vi "Main (429).vi"() -> ()   [LabVIEW 2023]
doc: "Use this template to build a simple state machine design pattern. Each state executes code and determines which state to transition to."
uses:
  Controls/State.ctl
  Controls/Data.ctl
  Controls/Database_Array.ctl
  Controls/Encoding.ctl
  <vilib>/Utility/error.llb/DialogType.ctl
  <userlib>/_OpenG.lib/array/array.llb/Remove Duplicates from 1D Array (I32)__ogtk.vi
  <userlib>/_OpenG.lib/array/array.llb/Sort 1D Array (I32)__ogtk.vi
  <userlib>/_OpenG.lib/array/array.llb/Search 1D Array (I32)__ogtk.vi
  <userlib>/_OpenG.lib/array/array.llb/Index 1D Array Elements (Variant)__ogtk.vi
  Libraries/Ballard_429_Parameter_ni/Ballard_429_Parameter_ni.lvlib
  Libraries/Aim_429_Parameter_ni/AIM_429_Parameter_ni.lvlib
panel:
  in  "Enable Large Schedules?":bool
  in  "Create Timestamp Channels?":bool
  in  "Use Octal Labels?":bool
  in  "formatting":enum16{"NIVeriStandAdd-Ons", "ni", "ni-AIM"}(ring)
  in  "Configure SelfTestBus?":bool
  out "Progress":string
  in  "Stop Button":bool
  in  "Generate XMLs":bool
  in  "Database Filepath (xlsx)":path
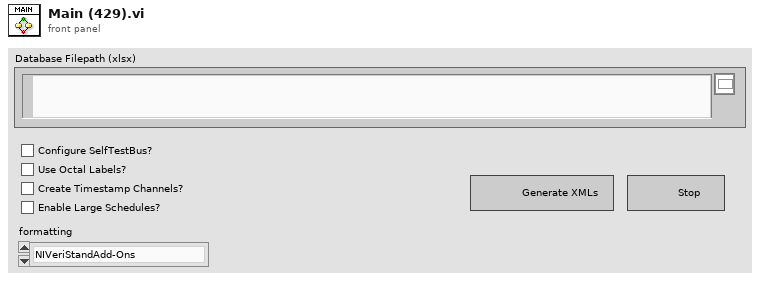
[diagram p1: front panel]
types:
  T1 = typedef "DialogType.ctl" = u16
  T2 = typedef "Data.ctl" = cluster{"Cores to Process Array":i32[], "All Parameters Array":T3[], "Filtered Parameter Array":T3[], "Core Number":i32, "Database Filepath (xlsx)":path, "Selected Self Test Channels":i32[], "formatting":enum16{"NIVeriStandAdd-Ons", "ni", "ni-AIM"}, "Use Octal Labels?":bool, "Create Timestamp Channels?":bool, "Configure SelfTestBus?":bool, "Enable Large Schedules?":bool}
  T3 = typedef "Database_Array.ctl" = cluster{"Core Number":i32, "Channel Number":i32, "Channel Name":string, "Channel Speed":i32, "Label Decimal":u32, "Label Name":string, "Min Rate (mS)":i32, "Max Rate (mS)":i32, "SDI":i32, "SSM":i32, "Create SDI":bool, "Create SSM":bool, "Create Parity":bool, "Parameter Name":string, "Start Bit":i32, "Number of Bits":i32, "Scale":string, "Offset":string, "Signed":bool, "Unit":string, "Encoding":T4, "Default Value":string}
  T4 = typedef "Encoding.ctl" = enum16{"BCD", "BNR", "Discrete"}
  T5 = typedef "State.ctl" = enum16{"Initialize", "Wait for Event", "Read Database File", "Get Core Data", "Write HW XML File", "Write Parameter XML File", "Exit"}
  T6 = enum8{"Enabled", "Disabled", "Disabled and Grayed Out"}
  T7 = enum32{"invalid app kind", "Development System", "Run Time System", "Student Edition", "Embedded LabVIEW", "Evaluation", "Custom"}
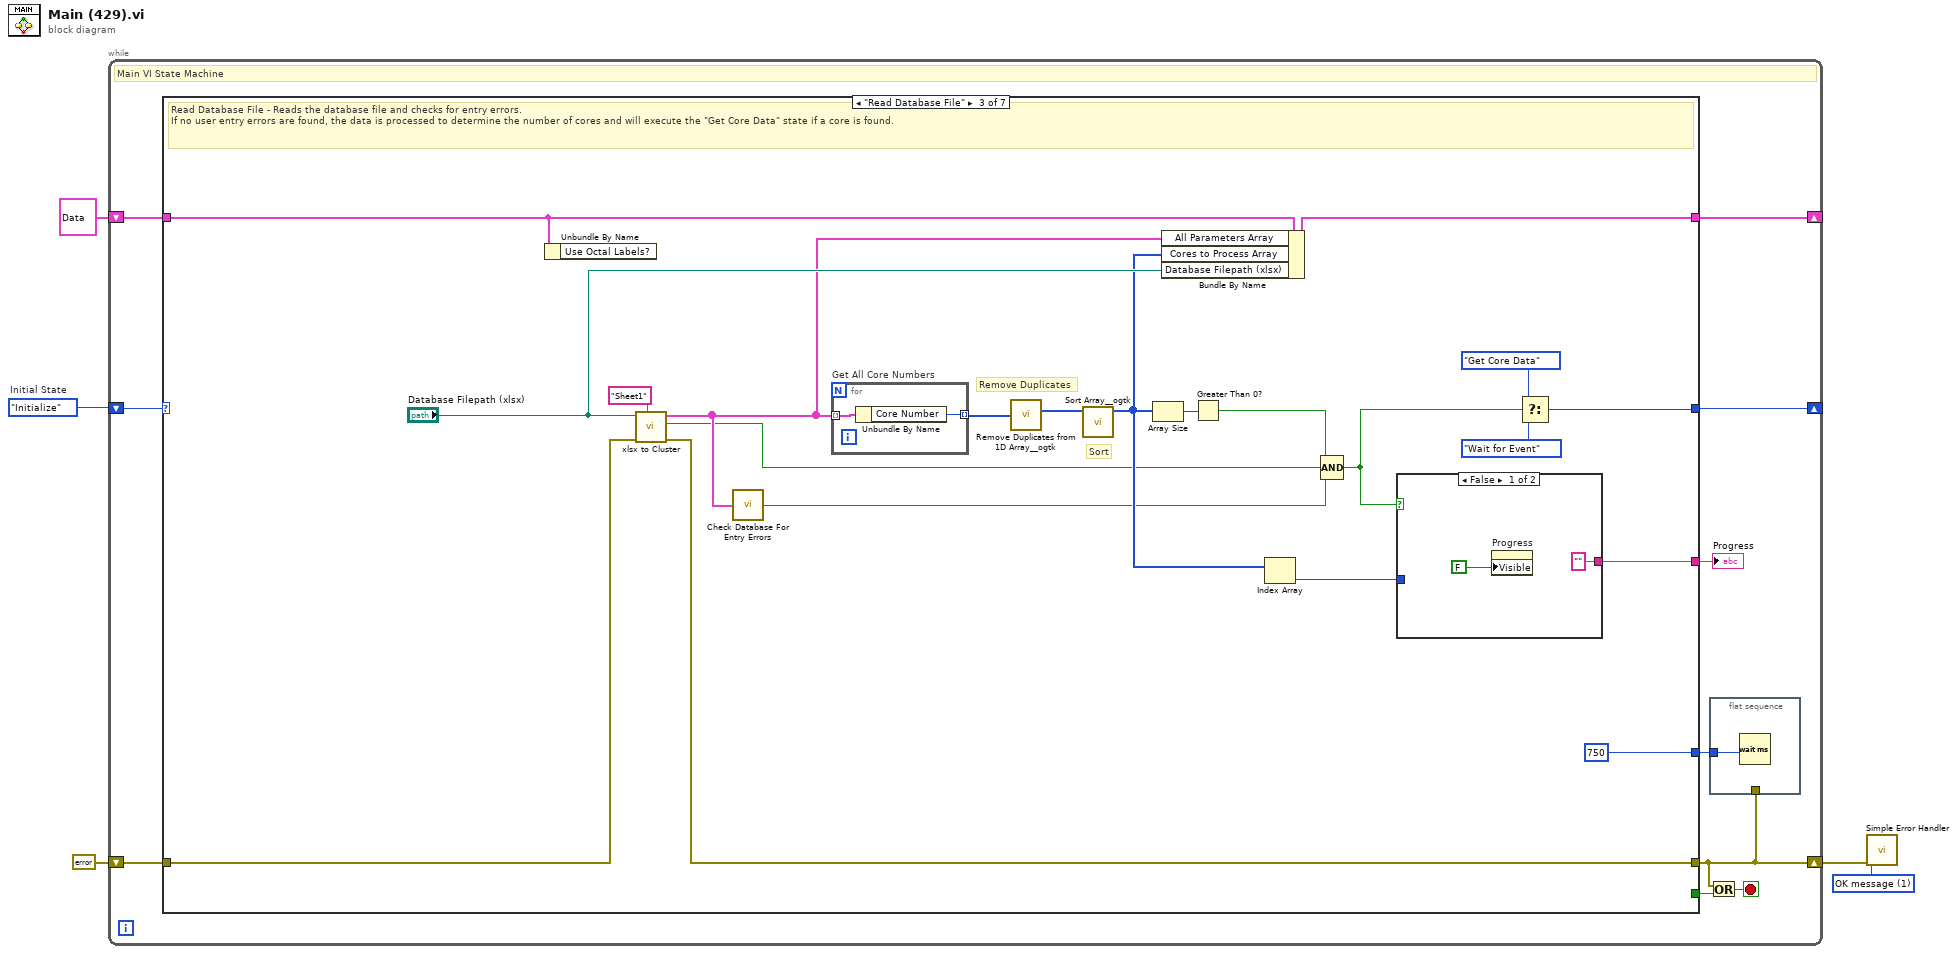
[diagram p0: block diagram]
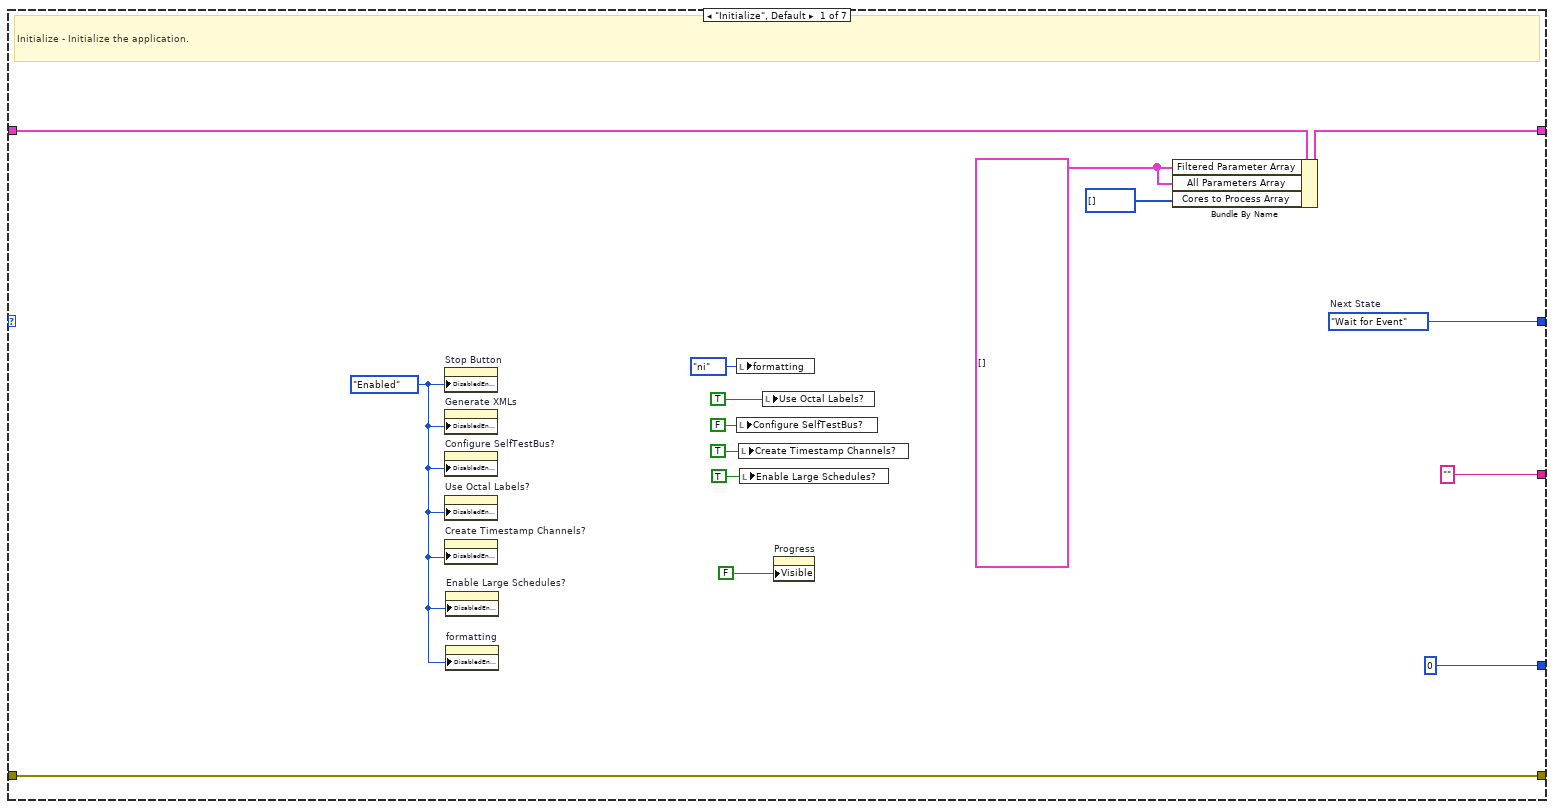
[diagram p2: hidden frame]
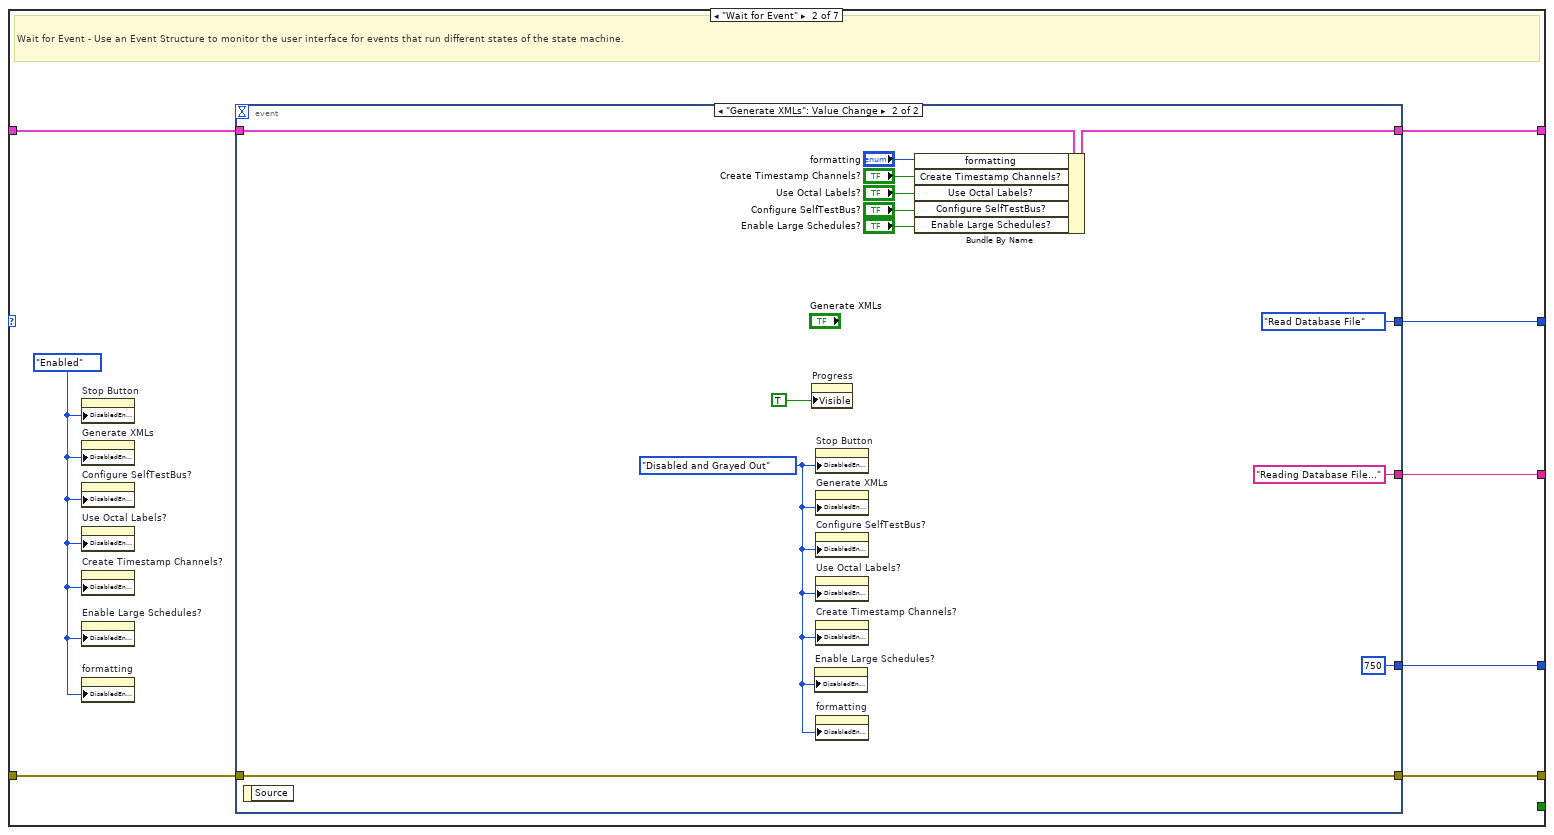
[diagram p3: hidden frame]
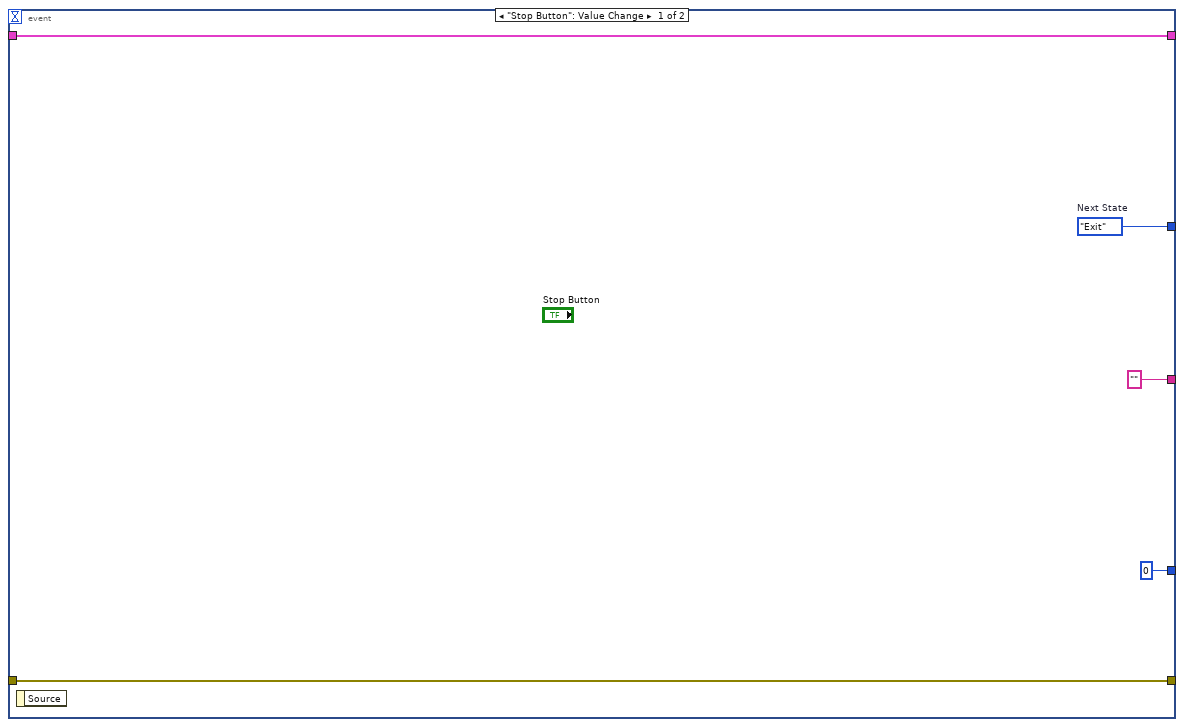
[diagram p4: hidden frame]
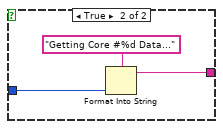
[diagram p5: hidden frame]
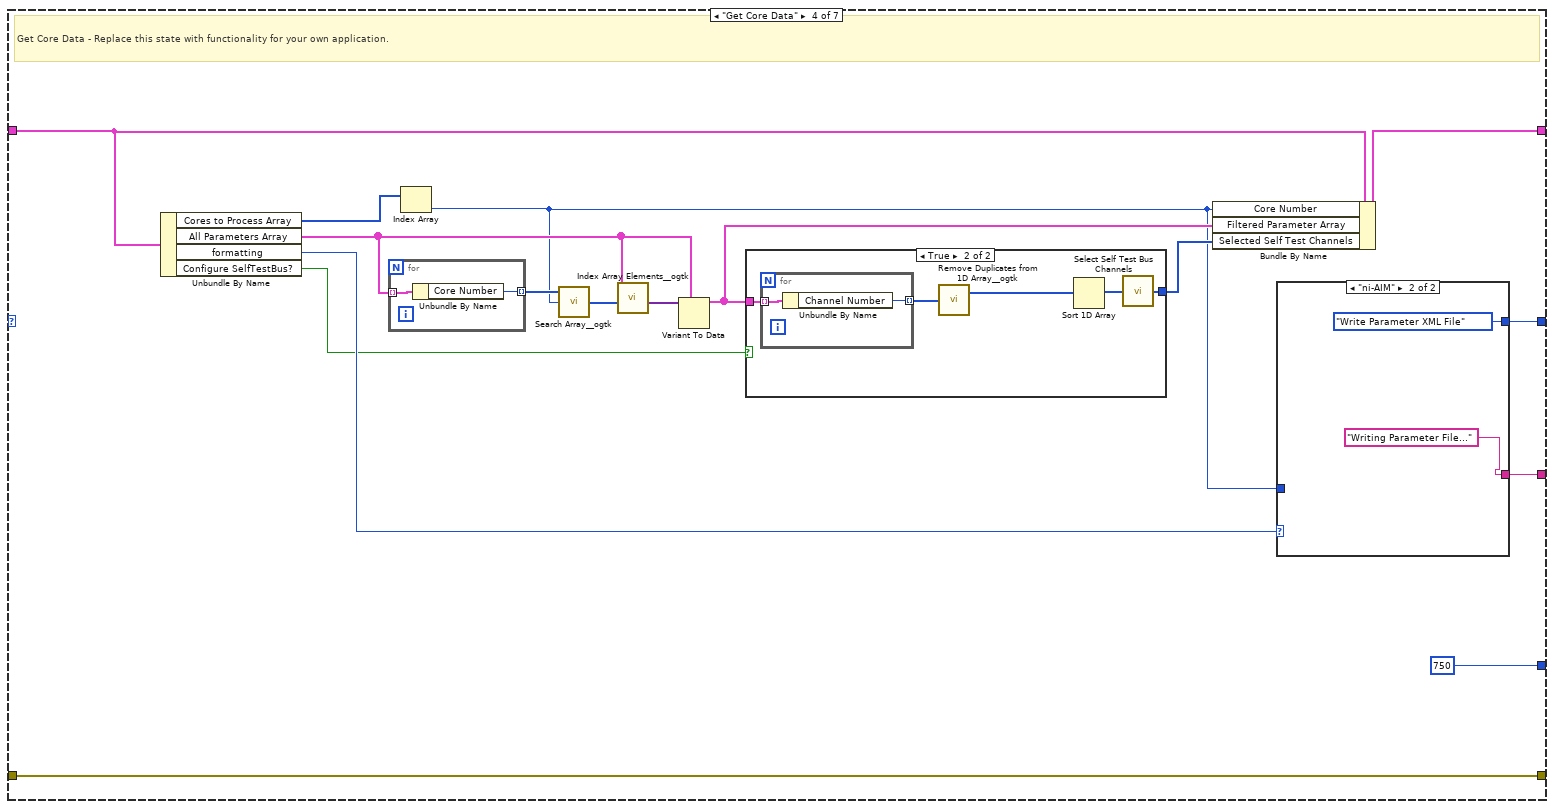
[diagram p6: hidden frame]
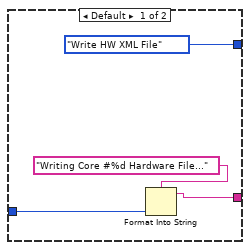
[diagram p7: hidden frame]
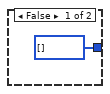
[diagram p8: hidden frame]
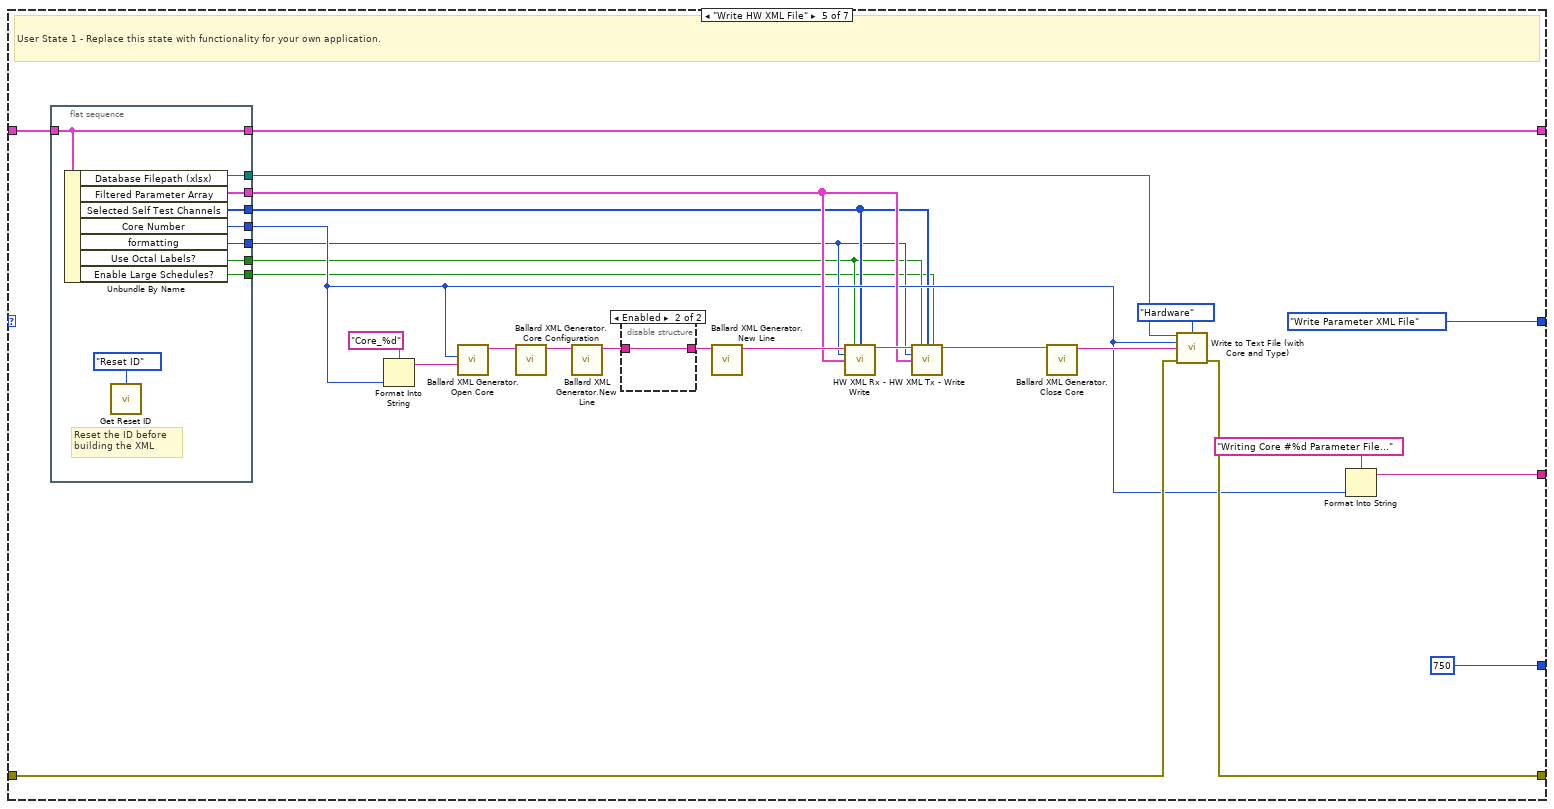
[diagram p9: hidden frame]
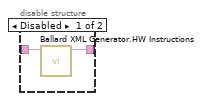
[diagram p10: hidden frame]
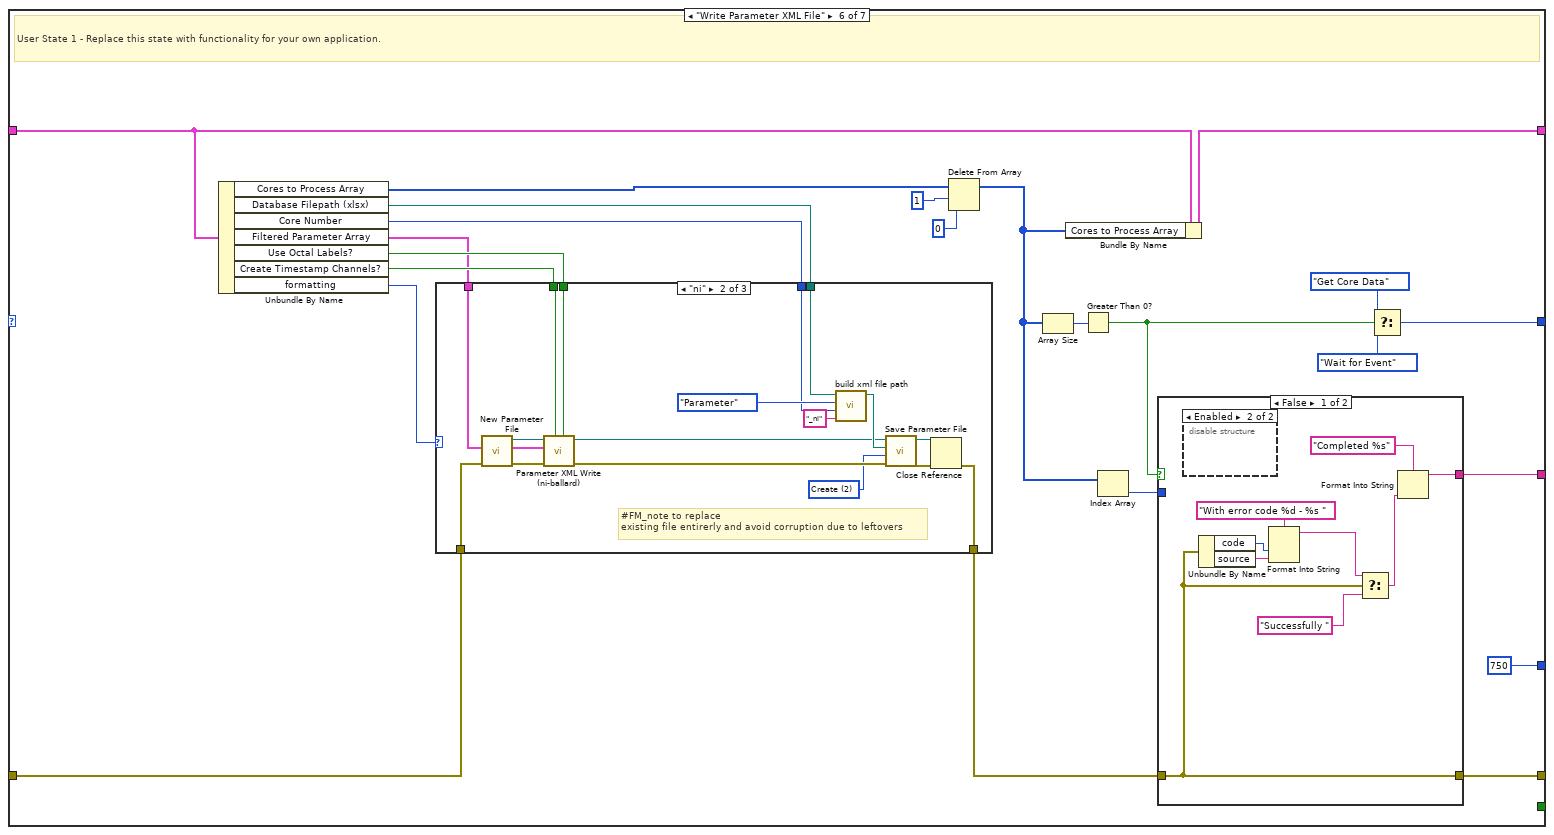
[diagram p11: hidden frame]
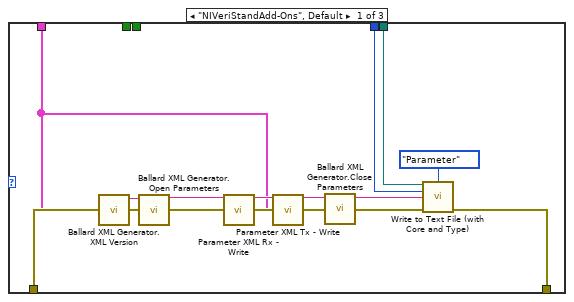
[diagram p12: hidden frame]
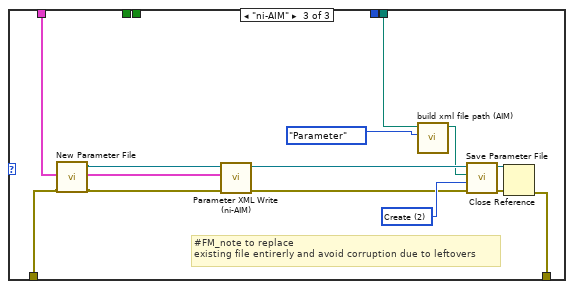
[diagram p13: hidden frame]
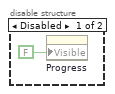
[diagram p14: hidden frame]
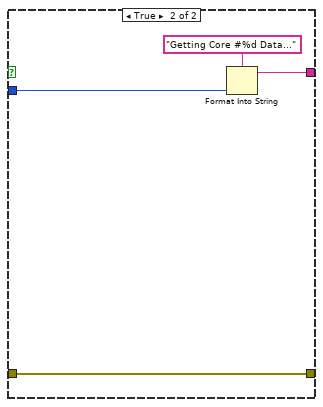
[diagram p15: hidden frame]
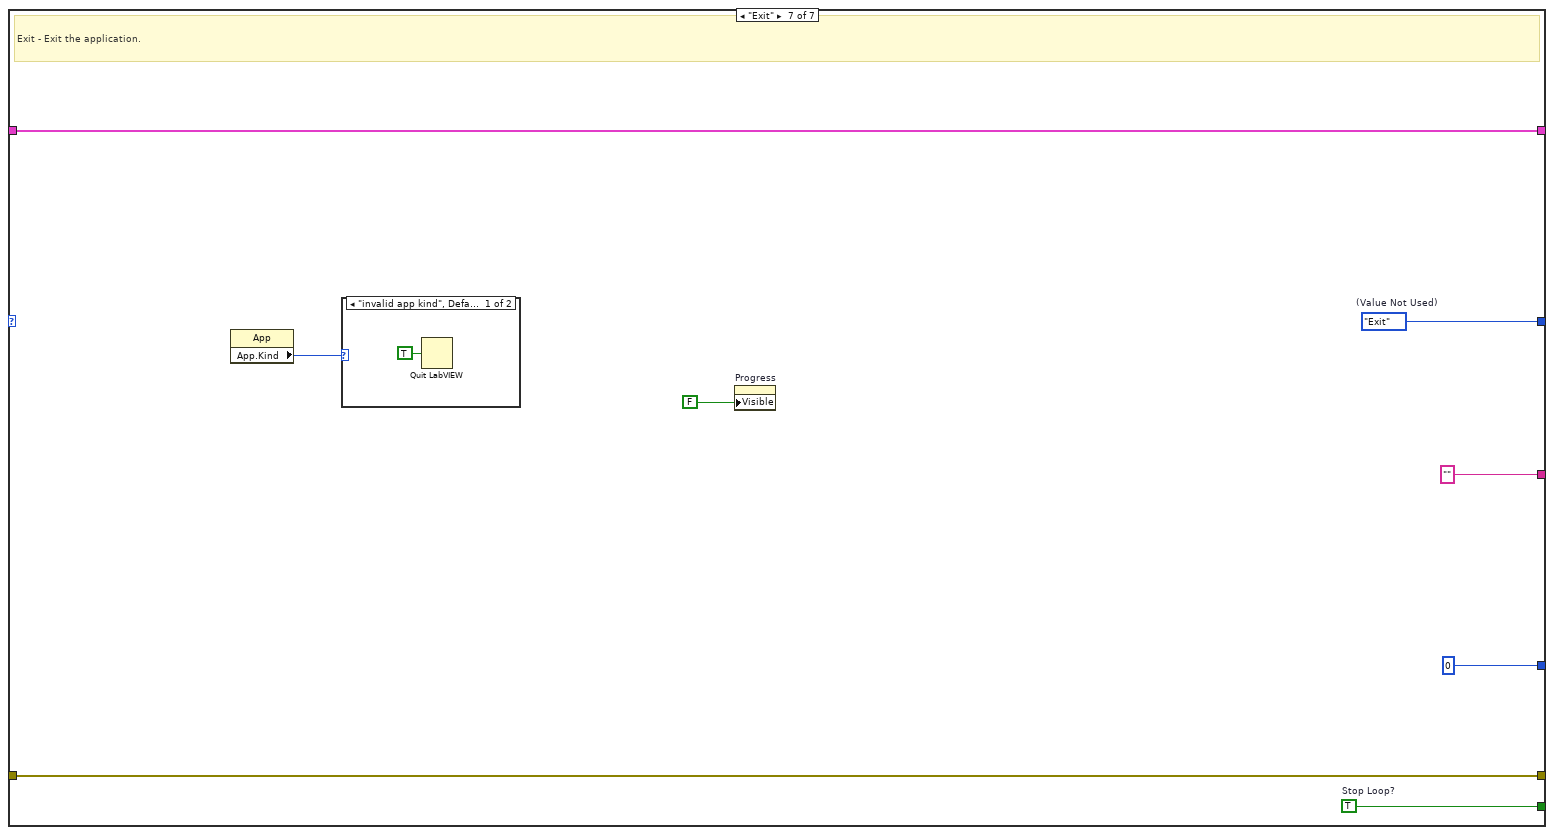
[diagram p16: hidden frame]
diagram:
  w1 = T1 1 items=["no dialog", "OK message", "continue or stop message", "OK message + warnings", "continue/stop + warnings"] ("type of dialog (OK msg:1)")
  w5 = State."Initialize"  # Initial State
  n1 = while {
    shift-right: [w14] -> _
    shift-left: w5 -> [w15]
    shift-right: [w12] -> _
    shift-left: T2 {"Cores to Process Array"=[], "All Parameters Array"=[], "Filtered Parameter Array"=[], "Core Number"=0, "Database Filepath (xlsx)"=path "C:/Users/jkreienh/Desktop/Preliminary Ballard Database Template.xlsx", "Selected Self Test Channels"=[], "formatting"=enum."NIVeriStandAdd-Ons", "Use Octal Labels?"=FALSE, "Create Timestamp Channels?"=FALSE, "Configure SelfTestBus?"=FALSE, "Enable Large Schedules?"=FALSE} ("Data") -> [w13]
    shift-right: [w7] -> w2
    shift-left: errorcluster {"status"=FALSE, "code"=0, "source"=""} ("error constant") -> [w11]
    stop <- w9 stop-if-true
    # "Main VI State Machine"
    n2 = case shown="\"Read Database File\"" w15 {
      tunnel: [w31 w39 w70 w95 State."Write Parameter XML File" ("Next State") w174 w241] -> w14
      tunnel: [_ _ _ _ _ _ w239] -> w10
      tunnel: w13 -> [w29 w38 w62 w99 w128 w171 w240]
      tunnel: [w28 w37 w74 w92 w127 w170 w240] -> w12
      tunnel: w11 -> [w30 w36 w67 w94 w131 w178 w238]
      tunnel: [w30 w35 w77 w94 w130 w160 w238] -> w7
      tunnel: ["" w34 w66 w87 w124 w167 ""] -> w8
      tunnel: [u32 0 ("milliseconds to wait") w33 u32 750 ("milliseconds to wait") u32 750 ("milliseconds to wait") u32 750 ("milliseconds to wait") u32 750 ("milliseconds to wait") u32 0 ("milliseconds to wait")] -> w6
      frame "Initialize", Default {
        w18 = T6."Enabled" ("Disabled")
        w26 = T3[] [] ("Parameter Array")
        w31 = State."Wait for Event"  # Next State
        # "Initialize - Initialize the application."
        n3 = property on="Stop Button" class="Bool"("DisabledEnum"=w18) -> ()  [unwired: 2 in, 2 out]
        n4 = property on="Generate XMLs" class="Bool"("DisabledEnum"=w18) -> ()  [unwired: 2 in, 2 out]
        n5 = property on="Configure SelfTestBus?" class="Bool (strict)"("DisabledEnum"=w18) -> ()  [unwired: 2 in, 2 out]
        n6 = property on="Use Octal Labels?" class="Bool (strict)"("DisabledEnum"=w18) -> ()  [unwired: 2 in, 2 out]
        n7 = property on="Create Timestamp Channels?" class="Bool (strict)"("DisabledEnum"=w18) -> ()  [unwired: 2 in, 2 out]
        n8 = property on="Enable Large Schedules?" class="Bool (strict)"("DisabledEnum"=w18) -> ()  [unwired: 2 in, 2 out]
        n9 = property on="formatting" class="Enum (strict)"("DisabledEnum"=w18) -> ()  [unwired: 2 in, 2 out]
        n10 = local write "formatting"(enum16{"NIVeriStandAdd-Ons", "ni", "ni-AIM"}."ni" ("formatting")) -> ()
        n11 = local write "Configure SelfTestBus?"(FALSE ("Configure SelfTestBus?")) -> ()
        n12 = local write "Create Timestamp Channels?"(TRUE ("Create Timestamp Channels?")) -> ()
        n13 = local write "Enable Large Schedules?"(TRUE ("Create Timestamp Channels?")) -> ()
        n14 = local write "Use Octal Labels?"(TRUE ("Use Octal Channel Names?")) -> ()
        n15 = property on="Progress" class="Str"("Visible"=FALSE) -> ()  [unwired: 2 in, 2 out]
        n16 = Bundle By Name(cluster=w29, "Filtered Parameter Array"=w26, "All Parameters Array"=w26, "Cores to Process Array"=i32[] [] ("Core Array")) -> (w28:T2)
      }
      frame "Wait for Event" {
        w32 = T6."Enabled" ("Disabled")
        # "Wait for Event - Use an Event Structure to monitor the user interface for events that run different states of the state machine."
        n17 = property on="Stop Button" class="Bool"("DisabledEnum"=w32) -> ()  [unwired: 2 in, 2 out]
        n18 = property on="Generate XMLs" class="Bool"("DisabledEnum"=w32) -> ()  [unwired: 2 in, 2 out]
        n19 = property on="Configure SelfTestBus?" class="Bool (strict)"("DisabledEnum"=w32) -> ()  [unwired: 2 in, 2 out]
        n20 = property on="Use Octal Labels?" class="Bool (strict)"("DisabledEnum"=w32) -> ()  [unwired: 2 in, 2 out]
        n21 = property on="Create Timestamp Channels?" class="Bool (strict)"("DisabledEnum"=w32) -> ()  [unwired: 2 in, 2 out]
        n22 = property on="Enable Large Schedules?" class="Bool (strict)"("DisabledEnum"=w32) -> ()  [unwired: 2 in, 2 out]
        n23 = property on="formatting" class="Enum (strict)"("DisabledEnum"=w32) -> ()  [unwired: 2 in, 2 out]
        n24 = event shown="[1] \"Generate XMLs\": Value Change" {
          selector: _ -> [_ _]
          dyn-events: _ -> [_ _]
          timeout: _ -> [_ _]
          tunnel: [w44 State."Read Database File" ("Next State")] -> w39
          tunnel: w38 -> [w43 w57]
          tunnel: [w43 w51] -> w37
          tunnel: w36 -> [w42 w56]
          tunnel: [w42 w56] -> w35
          tunnel: ["" "Reading Database File..."] -> w34
          tunnel: [u32 0 ("milliseconds to wait") u32 750 ("milliseconds to wait")] -> w33
          event "Stop Button": Value Change {
            w44 = State."Exit"  # Next State
            n25 = event-data() -> ()  [unwired: 1 in, 1 out]
          }
          event "Generate XMLs": Value Change {
            w45 = T6."Disabled and Grayed Out" ("Disabled")
            n26 = event-data() -> ()  [unwired: 1 in, 1 out]
            n27 = property on="Progress" class="Str"("Visible"=TRUE) -> ()  [unwired: 2 in, 2 out]
            n28 = property on="Enable Large Schedules?" class="Bool (strict)"("DisabledEnum"=w45) -> ()  [unwired: 2 in, 2 out]
            n29 = property on="Stop Button" class="Bool"("DisabledEnum"=w45) -> ()  [unwired: 2 in, 2 out]
            n30 = property on="Generate XMLs" class="Bool"("DisabledEnum"=w45) -> ()  [unwired: 2 in, 2 out]
            n31 = property on="Configure SelfTestBus?" class="Bool (strict)"("DisabledEnum"=w45) -> ()  [unwired: 2 in, 2 out]
            n32 = property on="Use Octal Labels?" class="Bool (strict)"("DisabledEnum"=w45) -> ()  [unwired: 2 in, 2 out]
            n33 = property on="Create Timestamp Channels?" class="Bool (strict)"("DisabledEnum"=w45) -> ()  [unwired: 2 in, 2 out]
            n34 = property on="formatting" class="Enum (strict)"("DisabledEnum"=w45) -> ()  [unwired: 2 in, 2 out]
            n35 = Bundle By Name(cluster=w57, "formatting"="formatting", "Create Timestamp Channels?"="Create Timestamp Channels?", "Use Octal Labels?"="Use Octal Labels?", "Configure SelfTestBus?"="Configure SelfTestBus?", "Enable Large Schedules?"="Enable Large Schedules?") -> (w51:T2)
          }
        }
      }
      frame "Read Database File" {
        # "Sort"
        # "Remove Duplicates"
        # "Read Database File - Reads the database file and checks for entry errors. \nIf no user entry errors are found, the data is processed to determine the number of cores and will execute the \"Get Core Data\" state if a core is found."
        n36 = Unbundle By Name(w62) -> ()  [unwired: 1 out]
        n37 = call "xlsx to Cluster.vi"("Excel._SheetName"="Sheet1", "Error (in)"=w67, "file path (dialog if empty)"="Database Filepath (xlsx)") -> ("Error (out)"=w77:errorcluster, "All Octal?"=w58:bool, "Parameter Array"=w68:T3[])  [unwired: 6 in]
        n38 = call "Check Database For Entry Errors.vi"("All Parameters Array"=w68) -> ("Database OK?"=w60:bool)  [unwired: 14 in]
        n39 = for "Get All Core Numbers" {
          tunnel: w68 -> [w85] mode=indexing
          tunnel: [w84] -> w76 mode=indexing
          n40 = Unbundle By Name(w85) -> ("Core Number"=w84:i32)
        }
        n41 = call-poly <userlib>:"Remove Duplicates from 1D Array__ogtk.vi"("Input Array"=w76) -> ("Output Array"=w75:i32[])  [unwired: 1 out]
        n42 = call-poly <userlib>:"Sort Array__ogtk.vi"("Array in"=w75) -> ("Sorted Array out"=w65:i32[])  [unwired: 9 in, 1 out]
        n43 = Array Size(array=w65) -> (size(s)=w73:i32)
        n44 = Bundle By Name(cluster=w62, "All Parameters Array"=w68, "Cores to Process Array"=w65, "Database Filepath (xlsx)"="Database Filepath (xlsx)") -> (w74:T2)
        n45 = Greater Than 0?(x=w73) -> (x > 0?=w61:bool)
        n46 = Index Array(array=w65) -> (element=w64:i32)  [unwired: 1 in]
        n47 = Compound Arithmetic op=AND(w61, w58, w60) -> (w59:bool)
        n48 = case shown="False" w59 {
          tunnel: ["" ("f") w82] -> w66
          tunnel: w64 -> [_ w83]
          frame False {
            n49 = property on="Progress" class="Str"("Visible"=FALSE) -> ()  [unwired: 2 in, 2 out]
          }
          frame True {
            n50 = Format Into String(format string="Getting Core #%d Data..." ("String"), w83) -> (resulting string=w82:string)  [unwired: 2 in, 1 out]
          }
        }
        n51 = Select(t=State."Get Core Data", s=w59, f=State."Wait for Event") -> (s? t:f=w70:T5)
      }
      frame "Get Core Data" {
        # "Get Core Data - Replace this state with functionality for your own application."
        n52 = Unbundle By Name(w99) -> ("Cores to Process Array"=w96:i32[], "All Parameters Array"=w98:T3[], "formatting"=w89:enum16{"NIVeriStandAdd-Ons", "ni", "ni-AIM"}, "Configure SelfTestBus?"=w86:bool)
        n53 = for {
          tunnel: w98 -> [w117] mode=indexing
          tunnel: [w116] -> w101 mode=indexing
          n54 = Unbundle By Name(w117) -> ("Core Number"=w116:i32)
        }
        n55 = Index Array(array=w96) -> (element=w88:i32)  [unwired: 1 in]
        n56 = call-poly <userlib>:"Search Array__ogtk.vi"("Array"=w101, "Element Data"=w88) -> ("Indices of Elements"=w100:i32[])  [unwired: 7 in]
        n57 = call-poly <userlib>:"Index Array Elements__ogtk.vi"("indices"=w100, "array"=w98) -> ("elements"=w97:variant[])  [unwired: 9 in]
        n58 = Variant To Data(type=w98, Variant=w97) -> (data=w91:T3[])  [unwired: 1 in, 1 out]
        n59 = case shown="True" w86 {
          tunnel: w91 -> [_ w112]
          tunnel: [i32[] [] ("Selected Channels") w109] -> w90
          frame False {
          }
          frame True {
            n60 = for {
              tunnel: [w115] -> w111 mode=indexing
              tunnel: w112 -> [w114] mode=indexing
              n61 = Unbundle By Name(w114) -> ("Channel Number"=w115:i32)
            }
            n62 = call-poly <userlib>:"Remove Duplicates from 1D Array__ogtk.vi"("Input Array"=w111) -> ("Output Array"=w113:i32[])  [unwired: 1 out]
            n63 = Sort 1D Array(array=w113) -> (sorted array=w110:i32[])
            n64 = call "Select Self Test Bus Channels.vi"("Channels"=w110) -> ("Selected Channels"=w109:i32[])  [unwired: 14 in]
          }
        }
        n65 = Bundle By Name(cluster=w99, "Core Number"=w88, "Filtered Parameter Array"=w91, "Selected Self Test Channels"=w90) -> (w92:T2)
        n66 = case shown="\"ni-AIM\"" w89 {
          tunnel: [State."Write HW XML File" State."Write Parameter XML File"] -> w95
          tunnel: w88 -> [w103 _]
          tunnel: [w102 "Writing Parameter File..." ("String")] -> w87
          frame Default {
            n67 = Format Into String(format string="Writing Core #%d Hardware File..." ("String"), w103) -> (resulting string=w102:string)  [unwired: 2 in, 1 out]
          }
          frame "ni-AIM" {
          }
        }
      }
      frame "Write HW XML File" {
        # "User State 1 - Replace this state with functionality for your own application."
        n68 = flat-sequence {
          tunnel: [w152] -> w133
          tunnel: w128 -> [w150]
          tunnel: [w150] -> w127
          tunnel: [w149] -> w126
          tunnel: [w148] -> w122
          tunnel: [w147] -> w121
          tunnel: [w146] -> w120
          tunnel: [w145] -> w119
          tunnel: [w144] -> w118
          frame #0 {
            # "Reset the ID before building the XML"
            n69 = Unbundle By Name(w150) -> ("Database Filepath (xlsx)"=w149:path, "Filtered Parameter Array"=w152:T3[], "Selected Self Test Channels"=w147:i32[], "Core Number"=w148:i32, "formatting"=w146:enum16{"NIVeriStandAdd-Ons", "ni", "ni-AIM"}, "Use Octal Labels?"=w145:bool, "Enable Large Schedules?"=w144:bool)
            n70 = call "Get Reset ID.vi"("Function"=enum16{"Get ID", "Reset ID"}."Reset ID") -> ()  [unwired: 14 in, 1 out]
          }
        }
        n71 = Format Into String(format string="Core_%d", w122) -> (resulting string=w134:string)  [unwired: 2 in, 1 out]
        n72 = call "Ballard XML Generator.Open Core.vi"("name"=w134, "id"=w122) -> ("string out"=w136:string)  [unwired: 9 in]
        n73 = call "Ballard XML Generator.Core Configuration.vi"("string in"=w136) -> ("string out"=w137:string)  [unwired: 10 in]
        n74 = call "Ballard XML Generator.New Line.vi"("string in"=w137) -> ("string out"=w138:string)  [unwired: 10 in]
        n75 = disable-structure shown="Enabled" {
          disable-tunnel: w138 -> [w154 w155]
          disable-tunnel: [w153 w155] -> w139
          frame Disabled {
            n76 = call "Ballard XML Generator.HW Instructions.vi"("string in"=w154) -> ("string out"=w153:string)  [unwired: 10 in]
          }
          frame Enabled {
          }
        }
        n77 = call "Ballard XML Generator.New Line.vi"("string in"=w139) -> ("string out"=w140:string)  [unwired: 10 in]
        n78 = call "HW XML Rx - Write.vi"("String (in)"=w140, "Use Octal Labels?"=w119, "Selected Channels"=w121, "formatting (NIVeriStandAdd-Ons)"=w120, "Parameter Array"=w133) -> ("String (out)"=w141:string)  [unwired: 10 in]
        n79 = call "HW XML Tx - Write.vi"("String (in)"=w141, "Use Octal Labels?"=w119, "Selected Channels"=w121, "Enable Large Schedules?"=w118, "formatting (NIVeriStandAdd-Ons)"=w120, "Parameter Array"=w133) -> ("String (out)"=w142:string)  [unwired: 9 in]
        n80 = call "Ballard XML Generator.Close Core.vi"("string in"=w142) -> ("string out"=w129:string)  [unwired: 10 in]
        n81 = call "Write to Text File (with Core and Type).vi"("Database Filepath (xlsx)"=w126, "Filetype"=enum16{"Hardware", "Parameter"}."Hardware", "Core"=w122, "Text"=w129, "Error (in)"=w131) -> ("Error (out)"=w130:errorcluster)  [unwired: 10 in]
        n82 = Format Into String(format string="Writing Core #%d Parameter File..." ("String"), w122) -> (resulting string=w124:string)  [unwired: 2 in, 1 out]
      }
      frame "Write Parameter XML File" {
        # "User State 1 - Replace this state with functionality for your own application."
        n83 = Unbundle By Name(w171) -> ("Cores to Process Array"=w172:i32[], "Database Filepath (xlsx)"=w169:path, "Core Number"=w166:i32, "Filtered Parameter Array"=w156:T3[], "Use Octal Labels?"=w159:bool, "Create Timestamp Channels?"=w158:bool, "formatting"=w157:enum16{"NIVeriStandAdd-Ons", "ni", "ni-AIM"})
        n84 = case shown="\"ni\"" w157 {
          tunnel: w178 -> [w185 w206 w218]
          tunnel: [w184 w205 w219] -> w161
          tunnel: w156 -> [w181 w190 w213]
          tunnel: w169 -> [w180 w201 w209]
          tunnel: w166 -> [w179 w200 _]
          tunnel: w159 -> [_ w191 _]
          tunnel: w158 -> [_ w192 _]
          frame "NIVeriStandAdd-Ons", Default {
            n85 = call "Ballard XML Generator.XML Version.vi"() -> ("string out"=w189:string)  [unwired: 11 in]
            n86 = call "Ballard XML Generator.Open Parameters.vi"("string in"=w189) -> ("string out"=w188:string)  [unwired: 10 in]
            n87 = call "Parameter XML Rx - Write.vi"("String (in)"=w188, "Parameter Array"=w181) -> ("String (out)"=w187:string)  [unwired: 13 in]
            n88 = call "Parameter XML Tx - Write.vi"("String (in)"=w187, "Parameter Array"=w181) -> ("String (out)"=w186:string)  [unwired: 13 in]
            n89 = call "Ballard XML Generator.Close Parameters.vi"("string in"=w186) -> ("string out"=w183:string)  [unwired: 10 in]
            n90 = call "Write to Text File (with Core and Type).vi"("Database Filepath (xlsx)"=w180, "Filetype"=enum16{"Hardware", "Parameter"}."Parameter", "Core"=w179, "Text"=w183, "Error (in)"=w185) -> ("Error (out)"=w184:errorcluster)  [unwired: 10 in]
          }
          frame "ni" {
            w193 = 2 items=["CreateNew"=1, "Create"=2, "Open"=3, "OpenOrCreate"=4, "Truncate"=5, "Append"=6] ("mode (Create)")
            # "#FM_note to replace \nexisting file entirerly and avoid corruption due to leftovers"
            n91 = call "New Parameter File.vi"("error in"=w206) -> ("error out"=w197:errorcluster, "new parameter file"=w198:refnum<k24>)  [unwired: 9 in]
            n92 = call "Parameter XML Write (ni-ballard).vi"("Use Octal Channel Names?"=w191, "Create TimeStamp Channels?"=w192, "error in"=w197, "Parameter Array"=w190, "parameter file in"=w198) -> ("error out"=w195:errorcluster, "parameter file out"=w196:refnum<k24>)  [unwired: 5 in]
            n93 = call "build xml file path.vi"("additional string(\"\")"="_ni" ("additional string(\"\")"), "Core"=w200, "Filetype"=enum16{"Hardware", "Parameter"}."Parameter", "Database Filepath in"=w201) -> ("xml path out"=w199:path)  [unwired: 7 in]
            n94 = call "Save Parameter File.vi"("error in"=w195, "mode (Create)"=w193, "XML path"=w199, "parameter file in"=w196) -> ("error out"=w204:errorcluster, "parameter file out"=w203:refnum<k24>)  [unwired: 5 in, 1 out]
            n95 = Close Reference(reference=w203, error in (no error)=w204) -> (error out=w205:errorcluster)
          }
          frame "ni-AIM" {
            w216 = 2 items=["CreateNew"=1, "Create"=2, "Open"=3, "OpenOrCreate"=4, "Truncate"=5, "Append"=6] ("mode (Create)")
            # "#FM_note to replace \nexisting file entirerly and avoid corruption due to leftovers"
            n96 = call "New Parameter File.vi"("error in"=w218) -> ("error out"=w210:errorcluster, "new parameter file"=w214:refnum<k24>)  [unwired: 9 in]
            n97 = call "Parameter XML Write (ni-AIM).vi"("error in"=w210, "Parameter Array"=w213, "parameter file in"=w214) -> ("error out"=w211:errorcluster, "parameter file out"=w212:refnum<k24>)  [unwired: 7 in]
            n98 = call "build xml file path (AIM).vi"("Filetype"=enum16{"Hardware", "Parameter"}."Parameter", "Database Filepath in"=w209) -> ("xml path out"=w207:path)  [unwired: 9 in]
            n99 = call "Save Parameter File.vi"("error in"=w211, "mode (Create)"=w216, "XML path"=w207, "parameter file in"=w212) -> ("error out"=w215:errorcluster, "parameter file out"=w217:refnum<k24>)  [unwired: 5 in, 1 out]
            n100 = Close Reference(reference=w217, error in (no error)=w215) -> (error out=w219:errorcluster)
          }
        }
        n101 = Delete From Array(array=w172, length=1, index=0) -> (array with subset deleted=w164:i32[])  [unwired: 1 out]
        n102 = Array Size(array=w164) -> (size(s)=w177:i32)
        n103 = Bundle By Name(cluster=w171, "Cores to Process Array"=w164) -> (w170:T2)
        n104 = Greater Than 0?(x=w177) -> (x > 0?=w165:bool)
        n105 = Index Array(array=w164) -> (element=w163:i32)  [unwired: 1 in]
        n106 = case shown="False" w165 {
          tunnel: [w227 w232] -> w167
          tunnel: w163 -> [_ w231]
          tunnel: w161 -> [w220 w230]
          tunnel: [w220 w230] -> w160
          frame False {
            n107 = disable-structure shown="Enabled" {
              frame Disabled {
                n108 = property on="Progress" class="Str"("Visible"=FALSE) -> ()  [unwired: 2 in, 2 out]
              }
              frame Enabled {
              }
            }
            n109 = Unbundle By Name(w220) -> ("code"=w225:i32, "source"=w224:string)
            n110 = Format Into String(format string="With error code %d - %s ", w225, w224) -> (resulting string=w222:string)  [unwired: 2 in, 1 out]
            n111 = Select(t=w222, s=w220, f="Successfully ") -> (s? t:f=w223:string)
            n112 = Format Into String(format string="Completed %s", w223) -> (resulting string=w227:string)  [unwired: 2 in, 1 out]
          }
          frame True {
            n113 = Format Into String(format string="Getting Core #%d Data..." ("String"), w231) -> (resulting string=w232:string)  [unwired: 2 in, 1 out]
          }
        }
        n114 = Select(t=State."Get Core Data" ("Next State"), s=w165, f=State."Wait for Event" ("Next State")) -> (s? t:f=w174:T5)
      }
      frame "Exit" {
        w239 = TRUE  # Stop Loop?
        w241 = State."Exit"  # (Value Not Used)
        # "Exit - Exit the application."
        n115 = property class="App"() -> ("App.Kind"=w234:T7)  [unwired: 2 in, 2 out]
        n116 = case shown="\"invalid app kind\", Default" w234 {
          frame "invalid app kind", Default {
            n117 = Quit LabVIEW(quit? (T)=TRUE) -> ()
          }
          frame "Development System" {
          }
        }
        n118 = property on="Progress" class="Str"("Visible"=FALSE) -> ()  [unwired: 2 in, 2 out]
      }
    }
    "Progress" <- w8
    n119 = Or(x=w7, y=w10) -> (x .or. y?=w9:bool)
    n120 = flat-sequence {
      tunnel: w7 -> [_]
      tunnel: w6 -> [w16]
      frame #0 {
        n121 = Wait (ms)(milliseconds to wait=w16) -> ()  [unwired: 1 out]
      }
    }
  }
  n122 = call <vilib>:"Simple Error Handler.vi"("type of dialog (OK msg:1)"=w1, "error in (no error)"=w2) -> ()  [unwired: 3 in, 5 out]
